vi "generate PWM Tag Lists.vi"(7 "input channel array":refnum<class "TBM channel.lvclass">[](array[class]), 8 "error in (no error)":errorcluster, 9 "Mappings in":T2 {"Line"."Parameters"."Voltage Config"."out terminal configuration (V)" items=["Default"=-1, "RSE"=10083, "Differential"=10106, "Pseudodifferential"=12529]; "Line"."Parameters"."Voltage Config"."in terminal configuration (V)" items=["Default"=-1, "RSE"=10083, "NRSE"=10078, "Differential"=10106, "Pseudodifferential"=12529]; "Line"."Parameters"."Current Config"."shunt resistor location" items=["default"=-1, "Internal"=10200, "External"=10167]; "Line"."Parameters"."Current Config"."input terminal configuration (C)" items=["default"=-1, "RSE"=10083, "NRSE"=10078, "Differential"=10106, "Pseudodifferential"=12529]; "Line"."Parameters"."RTD Config"."resistance configuration" items=["2-Wire"=2, "3-Wire"=3, "4-Wire"=4]; "Line"."Parameters"."RTD Config"."rtd type" items=["Pt3750"=12481, "Pt3851"=10071, "Pt3911"=12482, "Pt3916"=10069, "Pt3920"=10053, "Pt3928"=12483, "Custom"=10137]; "Line"."Parameters"."RTD Config"."current excitation source" items=["Internal"=10200, "External"=10167, "None"=10230]; "Line"."Parameters"."Thermocouple Config"."thermocouple type" items=["J"=10072, "K"=10073, "N"=10077, "R"=10082, "S"=10085, "T"=10086, "B"=10047, "E"=10055]; "Line"."Parameters"."Thermocouple Config"."cjc source" items=["Built-In"=10200, "Constant Value"=10116, "Channel"=10113]; "Line"."Parameters"."Strain Config"."bridge information"."strain configuration" items=["Full Bridge I"=10183, "Full Bridge II"=10184, "Full Bridge III"=10185, "Half Bridge I"=10188, "Half Bridge II"=10189, "Quarter Bridge I"=10271, "Quarter Bridge II"=10272]; "Line"."Parameters"."Strain Config"."bridge information"."voltage excitation source" items=["Internal"=10200, "External"=10167, "None"=10230]}, 10 "Measurement Type":T1, 11 "engine configuration in":refnum<class "engine configuration.lvclass">) -> (0 "Duty Cycle Index":i32=-1, 1 "Duty Cycle Array":string[](array[string]), 2 "Freq Index":i32=-1, 3 "Frequency Array":string[](array[string]), 5 "output channel array":refnum<class "TBM channel.lvclass">[](array[class]))   [LabVIEW 2015, in "DAQmx Module editor node.lvclass"]
doc: "This VI will be responsible for generating the two tag lists in the editor window for PWM signals (Frequency and Duty Cycle). This is a bit complicated by the bit that the item selected in one window can't exist in the other window."
uses:
  DAQmx Module editor node.lvclass
  Mappings.ctl
  module/configuration/Line.ctl
  <vilib>/NI/Tag Bus Module Framework/channel/TBM channel.lvclass
  module/configuration/Measurement Type.ctl
  module/configuration/Parameters.ctl
  Map.ctl
  <vilib>/NI/Module Execution Interface/Engine Configuration/engine configuration.lvclass
  <vilib>/NI/Tag Bus/tag/tag descriptor.lvclass/tag descriptor.ctl
  <vilib>/NI/Tag Bus Module Framework/channel/TBM channel.lvclass/TBM channel.ctl
  <vilib>/NI/Tag Bus/tag/write data type.vi
  <vilib>/NI/Tag Bus Module Framework/channel/Write channel classification.vi
  <vilib>/NI/Tag Bus/tag/tag descriptor.lvclass
  module/configuration/Daqmx Module configuration.lvclass
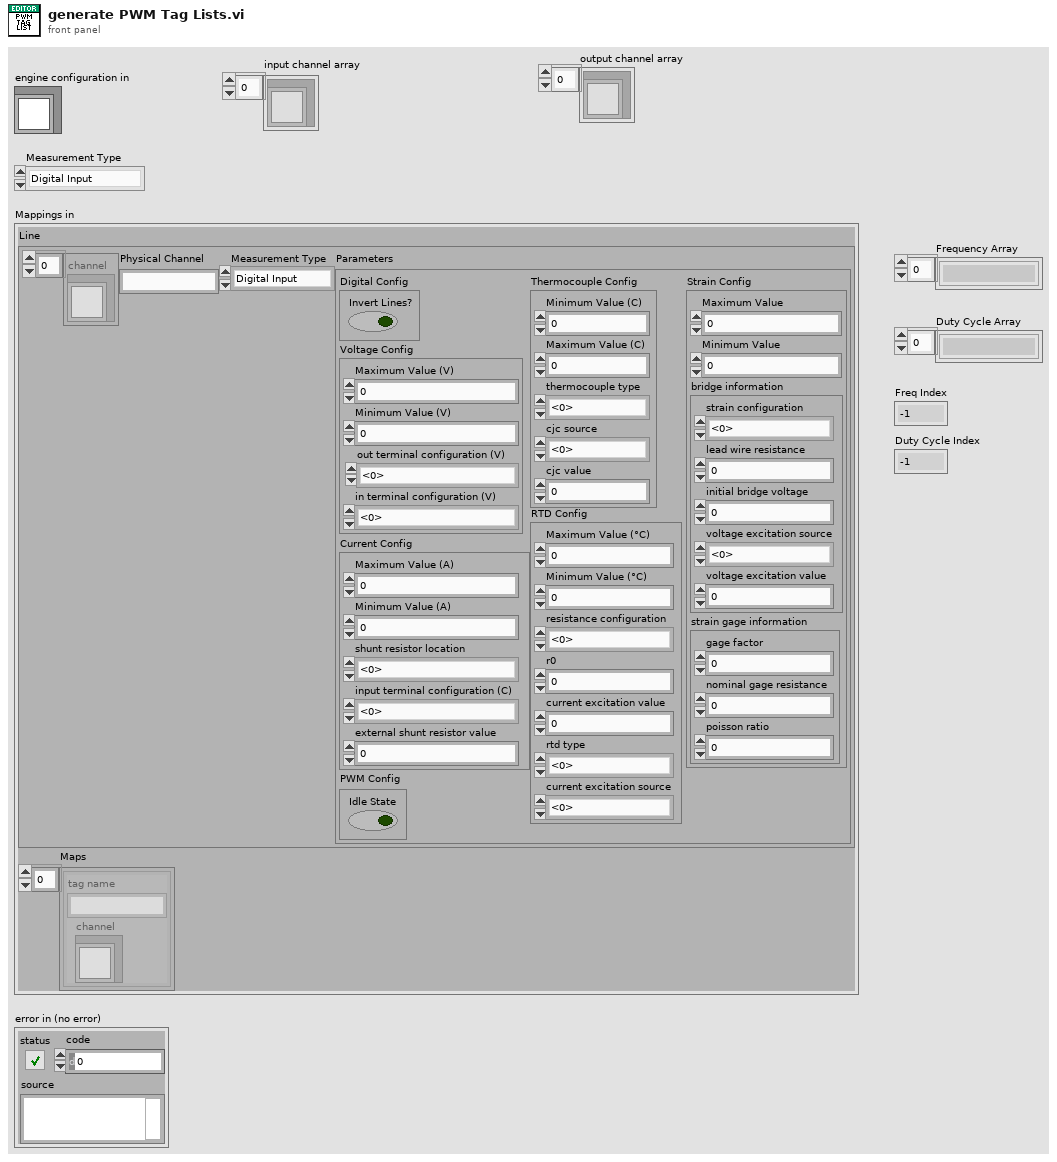
[diagram p1: front panel]
types:
  T1 = typedef "DAQmx Module Configuration.lvclass/Measurement Type.ctl" = enum16{"Digital Input", "Digital Output", "Voltage Input", "Voltage Output", "Current Input", "Current Output", "RTD", "Thermocouple", "Strain", "PWM"}
  T2 = typedef "DAQmx Module editor node.lvclass/Mappings.ctl" = cluster{"Line":T3, "Maps":T5[]}
  T3 = typedef "DAQmx Module Configuration.lvclass/Line.ctl" = cluster{"Channel Array":refnum<class "TBM channel.lvclass">[], "Physical Channel":string, "Measurement Type":T1, "Parameters":T4}
  T4 = typedef "DAQmx Module Configuration.lvclass/Parameters.ctl" = cluster{"Digital Config":cluster{"Invert Lines?":bool}, "Voltage Config":cluster{"Maximum Value (V)":dbl, "Minimum Value (V)":dbl, "in terminal configuration (V)":i32, "out terminal configuration (V)":i32}, "Current Config":cluster{"Maximum Value (A)":dbl, "Minimum Value (A)":dbl, "shunt resistor location":i32, "input terminal configuration (C)":i32, "external shunt resistor value":dbl}, "RTD Config":cluster{"Maximum Value (°C)":dbl, "Minimum Value (°C)":dbl, "resistance configuration":i32, "r0":dbl, "current excitation value":dbl, "rtd type":i32, "current excitation source":i32}, "Thermocouple Config":cluster{"Minimum Value (C)":dbl, "Maximum Value (C)":dbl, "thermocouple type":i32, "cjc source":i32, "cjc value":dbl}, "Strain Config":cluster{"Maximum Value":dbl, "Minimum Value":dbl, "bridge information":cluster{"strain configuration":i32, "lead wire resistance":dbl, "initial bridge voltage":dbl, "voltage excitation source":i32, "voltage excitation value":dbl}, "strain gage information":cluster{"gage factor":dbl, "nominal gage resistance":dbl, "poisson ratio":dbl}}, "PWM Config":cluster{"Idle State":bool}}
  T5 = typedef "DAQmx Module editor node.lvclass/Map.ctl" = cluster{"channel":refnum<class "TBM channel.lvclass">, "tag name":string}
  T6 = typedef "TBM channel.lvclass/channel classification.ctl" = enum16{"input data", "output data", "processing parameter", "processing result"}
  T7 = typedef "tag bus.lvlib/tag descriptor.lvclass/Data Type.ctl" = enum16{"Double", "Single", "I64", "I32", "I16", "I8", "U64", "U32", "U16", "U8", "Boolean", "String", "Array of Double", "Array of Single", "Array of I64", "Array of I32", "Array of I16", "Array of I8", "Array of U64", "Array of U32", "Array of U16", "Array of U8", "Array of Boolean", "Array of String"}
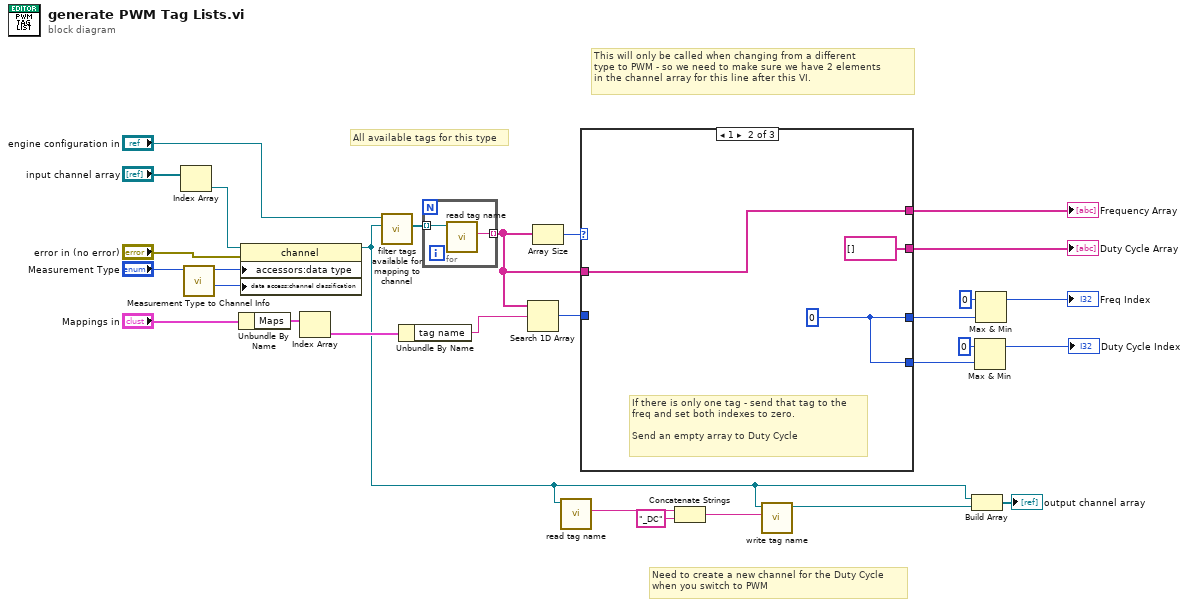
[diagram p0: block diagram]
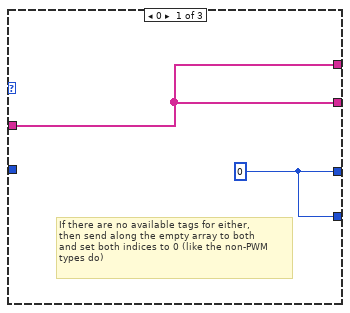
[diagram p2: hidden frame]
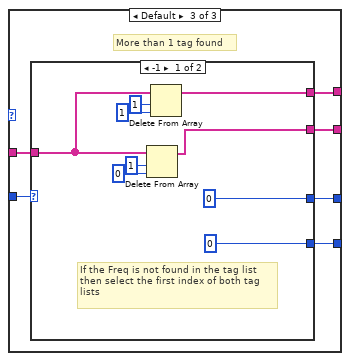
[diagram p3: hidden frame]
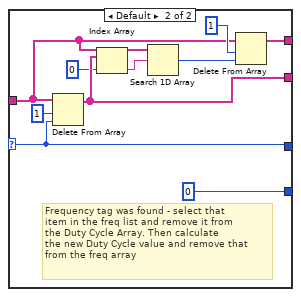
[diagram p4: hidden frame]
diagram:
  # "This will only be called when changing from a different\ntype to PWM - so we need to make sure we have 2 elements \nin the channel array for this line after this VI."
  # "Need to create a new channel for the Duty Cycle\nwhen you switch to PWM"
  # "All available tags for this type"
  n1 = Index Array(array="input channel array") -> (element=w18:refnum<class "TBM channel.lvclass">)  [unwired: 1 in]
  n2 = call "Measurement Type to Channel Info.vi"("Measurement Type"="Measurement Type") -> ("channel classification"=w24:T6, "Data Type"=w23:T7)  [unwired: 8 in]
  n3 = Unbundle By Name("Mappings in") -> ("Maps"=w27:T5[])
  n4 = property class="channel"(reference=w18, error in="error in (no error)", "accessors:data type"=w23, "data access:channel classification"=w24) -> (reference out=w12:refnum<class "TBM channel.lvclass">)  [unwired: 1 out]
  n5 = Index Array(array=w27) -> (element=w26:T5)  [unwired: 1 in]
  n6 = call-dynamic "filter tags available for mapping to channel.vi"("channel to map to"=w12, "engine configuration in"="engine configuration in") -> ("filtered tags"=w22:refnum<class "tag descriptor.lvclass">[])  [unwired: 8 in, 1 out]
  n7 = Unbundle By Name(w26) -> ("tag name"=w29:string)
  n8 = for {
    tunnel: w22 -> [w31] mode=indexing
    tunnel: [w30] -> w9 mode=indexing
    n9 = call <vilib>:"read tag name.vi"("system tag in"=w31) -> ("name"=w30:string)  [unwired: 8 in, 2 out]
  }
  n10 = Search 1D Array(1D array=w9, element=w29) -> (index of element=w21:i32)  [unwired: 1 in]
  n11 = Array Size(array=w9) -> (size(s)=w10:i32)
  n12 = call <vilib>:"read tag name.vi"("system tag in"=w12) -> ("name"=w15:string)  [unwired: 8 in, 2 out]
  n13 = case shown="1" w10 {
    tunnel: w21 -> [_ _ w42]
    tunnel: [w33 w36 w41] -> w3
    tunnel: [w33 w36 w40] -> w4
    tunnel: w9 -> [w32 w35 w39]
    tunnel: [w32 w35 w38] -> w8
    tunnel: [w32 string[] [] w37] -> w7
    frame 0 {
      w33 = 0
      # "If there are no available tags for either,\nthen send along the empty array to both\nand set both indices to 0 (like the non-PWM\ntypes do)"
    }
    frame 1 {
      w36 = 0
      # "If there is only one tag - send that tag to the \nfreq and set both indexes to zero.\n\nSend an empty array to Duty Cycle"
    }
    frame Default {
      # "More than 1 tag found"
      n14 = case shown="-1" w42 {
        selector: w42 -> [_ w57]
        tunnel: [0 ("index of element") 0 ("index of element")] -> w41
        tunnel: [0 ("index of element") w57] -> w40
        tunnel: w39 -> [w45 w56]
        tunnel: [w44 w58] -> w38
        tunnel: [w43 w55] -> w37
        frame -1 {
          # "If the Freq is not found in the tag list\nthen select the first index of both tag \nlists"
          n15 = Delete From Array(array=w45, length=1, index=0) -> (array with subset deleted=w43:string[])  [unwired: 1 out]
          n16 = Delete From Array(array=w45, length=1, index=1) -> (array with subset deleted=w44:string[])  [unwired: 1 out]
        }
        frame Default {
          # "Frequency tag was found - select that\nitem in the freq list and remove it from\nthe Duty Cycle Array. Then calculate\nthe new Duty Cycle value and remove that \nfrom the freq array"
          n17 = Delete From Array(array=w56, length=1, index=w57) -> (array with subset deleted=w55:string[])  [unwired: 1 out]
          n18 = Index Array(array=w55, index=0) -> (element=w53:string)
          n19 = Search 1D Array(1D array=w56, element=w53) -> (index of element=w52:i32)  [unwired: 1 in]
          n20 = Delete From Array(array=w56, length=1, index=w52) -> (array with subset deleted=w58:string[])  [unwired: 1 out]
        }
      }
    }
  }
  "Frequency Array" <- w8
  "Duty Cycle Array" <- w7
  n21 = Concatenate Strings(w15, "_DC" ("string")) -> (w13:string)
  n22 = call <vilib>:"write tag name.vi"("name"=w13, "system tag in"=w12) -> ("system tag out"=w11:refnum<class "TBM channel.lvclass">)  [unwired: 8 in, 1 out]
  n23 = Build Array(w12, w11) -> (→"output channel array":refnum<class "TBM channel.lvclass">[])
  n24 = Max & Min(x=0 ("f"), y=w3) -> (max(x,y)=→"Duty Cycle Index":i32)  [unwired: 1 out]
  n25 = Max & Min(x=0 ("f"), y=w4) -> (max(x,y)=→"Freq Index":i32)  [unwired: 1 out]
